vi "VM - Variable Attribute.vi"(7 "VC Handle":T2=-1, 8 "error in":errorcluster, 9 "cmd (read)":enum16{"read", "write"}(ring), 10 "Attribute in":string, 11 "name_spec":string) -> (0 "error out":errorcluster, 1 "DBL value":dbl, 2 "Attribute out":string, 3 "dup name_spec":string, 4 "type code":u32, 6 "writer ID":u32)   [LabVIEW 2021]
doc: "This VI reads or writes a variable attribute. You can use this VI to associate arbitrary data with a variable and store it as an attribute. An attribute is stored as a string; if any other type is desired for the attribute, convert it to or from a string before passing or after reading. Refer to the VI help for more details.\n\n<b>VC Handle</b> specifies the handle of the variable context. To operate on a global variable, pass -1 to this input. This input is ignored if the <b>name_spec</b> control refers to a variable by an alias.\n\n<b>name_spec</b> is the name specifier of the desired variable. Usually, it is merely a variable name; however, its generic format is '[name][=alias]', where either 'name' or '=alias' can be omitted but not both.\n\n<b>cmd</b> control specifies the action to be performed. Possible actions are 'read' and 'write'.\n\n<b>writer ID</b> indicator returns the ID of the writer for the most recent value.\n\n<b>type code</b> indicator returns the variable data type code. If the variable type is DBL Scalar (type code 1), <b>DBL value</b> indicator returns the actual variable value.\n\n::: CalcExpress Toolkit :::\nCopyright (c) 2000-2026 Konstantin Shifershteyn. All rights reserved."
uses:
  cetypes.llb/VarMan Variable Context Handle.ctl
  cetypes.llb/VarMan Error Code.ctl
  cersrc/celveng32.dll
panel:
  out "err code":T1 items=["No error", "Invalid variable type", "Variable not found", "Variable already exists", "Invalid context handle", "Input error", "Invalid data format", "No history attached", "History already attached", "Invalid history parameters", "Wrong variable name", "Wrong alias name", "Non-unique alias", "Alias not found", "No alias associated", "Alias already associated", "Wrong context name", "Non-unique context name", "Context name not found", "Invalid parameter", "Generic error", "Memory Full", "Unrecognized LV error", "Unknown error code"]
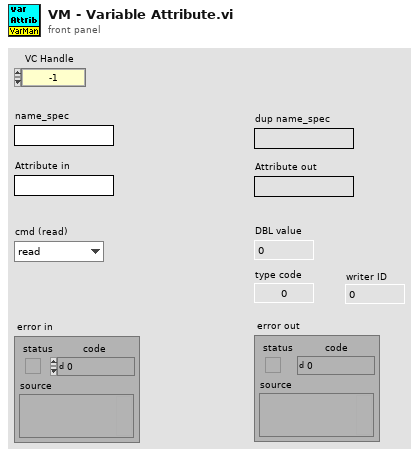
[diagram p1: front panel]
types:
  T1 = typedef "VarMan Error Code.ctl" = u16
  T2 = typedef "VarMan Variable Context Handle.ctl" = i32
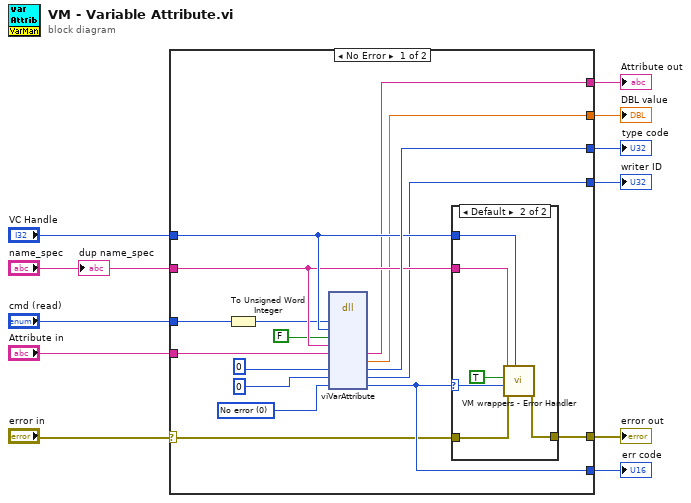
[diagram p0: block diagram]
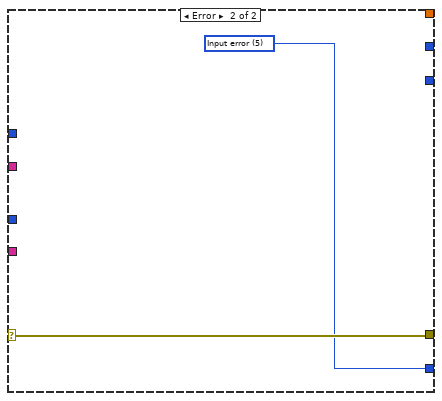
[diagram p3: hidden frame]
diagram:
  n1 = case shown="No Error" "error in" {
    selector: "error in" -> [w14 w36]
    tunnel: [w27 w36] -> w11
    tunnel: [w26 _] -> w10
    tunnel: "cmd (read)" -> [w25 _]
    tunnel: "VC Handle" -> [w24 _]
    tunnel: "name_spec" -> [w23 _]
    tunnel: [w22 _] -> w6
    tunnel: "Attribute in" -> [w21 _]
    tunnel: [w19 _] -> w4
    tunnel: [w18 w35] -> w3
    tunnel: [w13 _] -> w1
    frame No Error {
      w17 = T1 0 items=["No error", "Invalid variable type", "Variable not found", "Variable already exists", "Invalid context handle", "Input error", "Invalid data format", "No history attached", "History already attached", "Invalid history parameters", "Wrong variable name", "Wrong alias name", "Non-unique alias", "Alias not found", "No alias associated", "Alias already associated", "Wrong context name", "Non-unique context name", "Context name not found", "Invalid parameter", "Generic error", "Memory Full", "Unrecognized LV error", "Unknown error code"] ("err code")
      n2 = To Unsigned Word Integer(number=w25) -> (unsigned 16bit integer=w12:u16)
      n3 = dll-call lib="C:/LV Projects/CalcExpress 40 LV2021/vi.lib/addons/CalcExpress/cersrc/celveng*.dll" fn="viVarAttribute"("cmd"=w12, "vch"=w24, "gbl"=FALSE, "name"=w23, "attrib"=w21, "type"=u32 0 ("type code"), "writerID"=u32 0 ("type code"), "errc"=w17) -> ("attrib"=w22:string, "dblval"=w19:dbl, "type"=w26:u32, "writerID"=w13:u32, "errc"=w18:T1)  [unwired: 9 in, 2 out]
      n4 = case shown="Default" w18 {
        selector: w18 -> [_ w30]
        tunnel: [w28 w34] -> w27
        tunnel: w23 -> [_ w32]
        tunnel: w24 -> [_ w31]
        tunnel: w14 -> [w28 w29]
        frame 0 {
        }
        frame Default {
          n5 = call "VM wrappers - Error Handler.vi"("VC Handle"=w31, "error before"=w29, "VarMan error"=w30, "show name spec (F)"=TRUE, "name spec"=w32) -> ("error out"=w34:errorcluster)  [unwired: 5 in, 1 out]
        }
      }
    }
    frame Error {
      w35 = T1 5 items=["No error", "Invalid variable type", "Variable not found", "Variable already exists", "Invalid context handle", "Input error", "Invalid data format", "No history attached", "History already attached", "Invalid history parameters", "Wrong variable name", "Wrong alias name", "Non-unique alias", "Alias not found", "No alias associated", "Alias already associated", "Wrong context name", "Non-unique context name", "Context name not found", "Invalid parameter", "Generic error", "Memory Full", "Unrecognized LV error", "Unknown error code"] ("err code")
    }
  }
  "error out" <- w11
  "Attribute out" <- w6
  "err code" <- w3
  "type code" <- w10
  "DBL value" <- w4
  "writer ID" <- w1
  "dup name_spec" <- "name_spec"
